vi "Test MQTT-3.1.4-2.vi"(8 "error in (no error)":errorcluster, 11 "Connection Config":refnum<class "Connection.lvclass">) -> (0 "error out":errorcluster, 3 "Connection Config dup":refnum<class "Connection.lvclass">)   [LabVIEW 2013]
uses:
  <vilib>/LabVIEW Open Source Project/MQTT Control Packets/Control Packets/CONNECT/CONNECT.lvclass
  <vilib>/LabVIEW Open Source Project/MQTT Control Packets/Control Packets/ControlPacket/ControlPacket.lvclass
  <vilib>/addons/_JKI Toolkits/Caraya/classes/Test/Test.lvclass
  <vilib>/addons/_JKI Toolkits/Caraya/classes/Assert/Assert.lvclass
  <vilib>/LabVIEW Open Source Project/MQTT Control Packets/Control Packets/DISCONNECT/DISCONNECT.lvclass
  <vilib>/LabVIEW Open Source Project/MQTT Control Packets/Control Packets/CONNACK/CONNACK.lvclass
  <vilib>/LabVIEW Open Source Project/MQTT Control Packets/Control Packets/CONNACK/Connect Return Code -- enum.ctl
  <vilib>/LabVIEW Open Source Project/Connection/Connection/Connection.lvclass
  <vilib>/LabVIEW Open Source Project/MQTT Connection/MQTT_Connection/Connection/Connection.lvclass
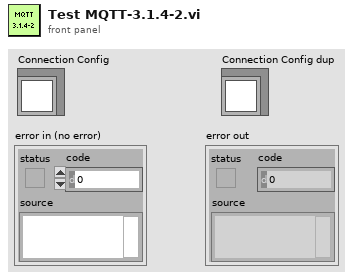
[diagram p1: front panel]
types:
  T1 = typedef "MQTT_Control_Packets.lvlib/CONNACK.lvclass/Connect Return Code -- enum.ctl" = enum16{"Connection accepted", "Unacceptable protocol version", "Identifier Rejected", "Server Unavailable", "Bad Username or Password", "Not Authorized"}
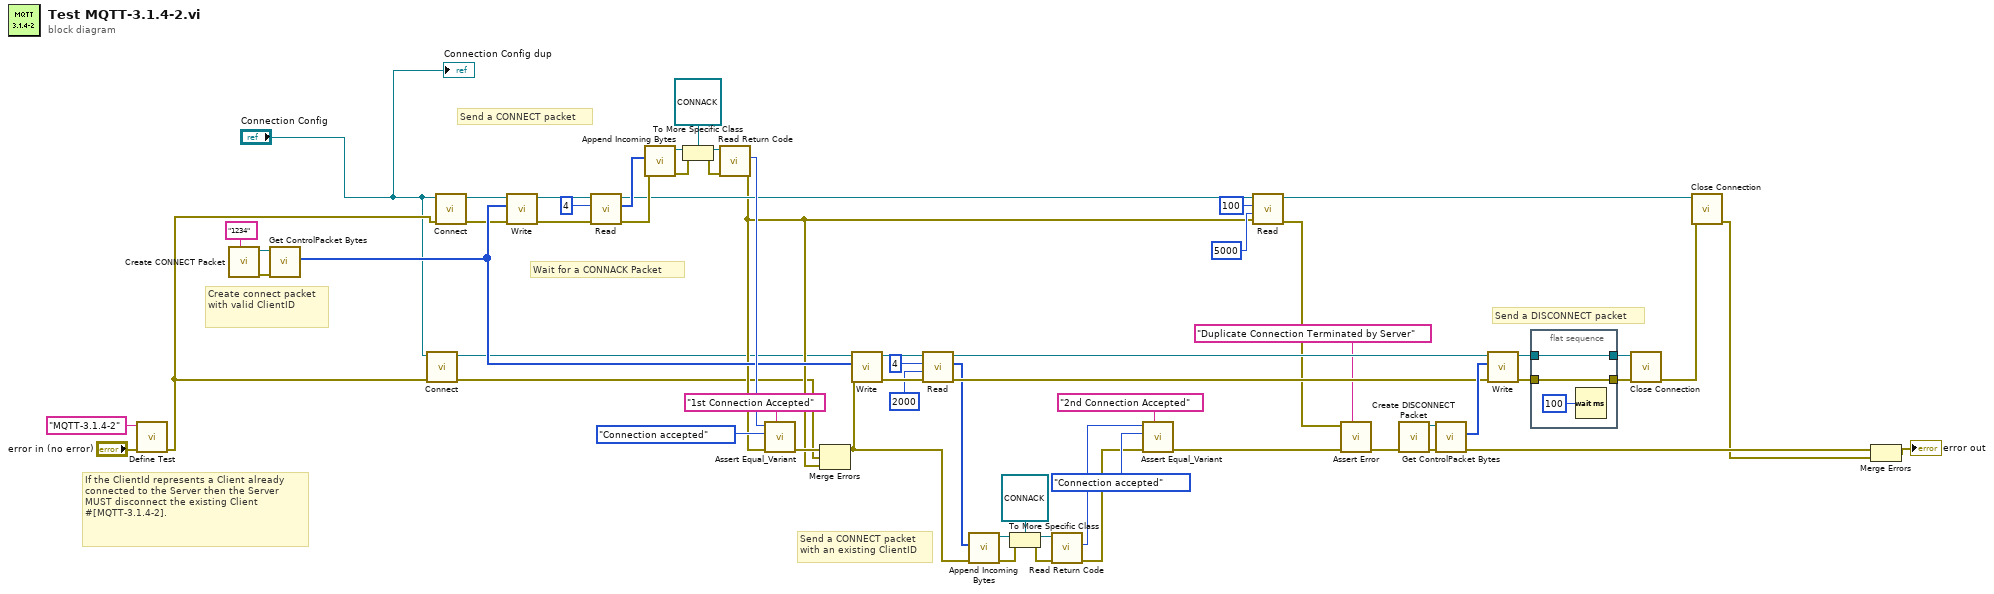
[diagram p0: block diagram]
diagram:
  # "Send a CONNECT packet\nwith an existing ClientID"
  # "If the ClientId represents a Client already connected to the Server then the Server MUST disconnect the existing Client #[MQTT-3.1.4-2]."
  # "Send a DISCONNECT packet"
  # "Wait for a CONNACK Packet"
  # "Create connect packet with valid ClientID"
  # "Send a CONNECT packet"
  n1 = call <vilib>:"Define Test.vi"("error in (no error)"="error in (no error)", "Label (VI Title)"="MQTT-3.1.4-2") -> ("error out"=w7:errorcluster)  [unwired: 9 in]
  n2 = call <vilib>:"Create CONNECT Packet.vi"("Client ID (empty: generate new)"="1234") -> ("error out"=w62:errorcluster, "CONNECT"=w63:refnum<class "CONNECT.lvclass">)  [unwired: 8 in, 1 out]
  n3 = call <vilib>:"Get ControlPacket Bytes.vi"("error in (no error)"=w62, "ControlPacket"=w63) -> ("Bytes Stream"=w38:u8[])  [unwired: 6 in, 3 out]
  n4 = call <vilib>:"Connect.vi"("error in (no error)"=w7, "Connection in"="Connection Config") -> ("error out"=w10:errorcluster, "Connection out"=w11:refnum<class "Connection.lvclass">)  [unwired: 8 in]
  n5 = call <vilib>:"Connect.vi"("error in (no error)"=w7, "Connection in"="Connection Config") -> ("error out"=w8:errorcluster, "Connection out"=w9:refnum<class "Connection.lvclass">)  [unwired: 8 in]
  n6 = call <vilib>:"Write.vi"("error in (no error)"=w8, "Bytes"=w38, "Connection in"=w9) -> ("error out"=w42:errorcluster, "Connection"=w43:refnum<class "Connection.lvclass">)  [unwired: 7 in]
  n7 = call <vilib>:"Read.vi"("error in (no error)"=w42, "bytes to read (100)"=4 ("bytes to read"), "TCPConnection in"=w43) -> ("error out"=w39:errorcluster, "Bytes"=w41:u8[], "TCPConnection out"=w28:refnum<class "Connection.lvclass">)  [unwired: 4 in, 2 out]
  n8 = call <vilib>:"Append Incoming Bytes.vi"("error in (no error)"=w39, "Incoming Packets"=w41) -> ("error out"=w45:errorcluster, "ControlPacket"=w51:refnum<class "ControlPacket.lvclass">)  [unwired: 6 in, 2 out]
  n9 = To More Specific Class(target class=refnum<class "CONNACK.lvclass"> refnum ("CONNACK"), reference=w51, error in=w45) -> (specific class reference=w50:refnum<class "CONNACK.lvclass">, error out=w46:errorcluster)
  n10 = call <vilib>:"Read Return Code.vi"("error in (no error)"=w46, "CONNACK in"=w50) -> ("error out"=w12:errorcluster, "Return Code"=w48:T1)  [unwired: 7 in, 1 out]
  n11 = call <vilib>:"Assert Equal_Variant.vi"("Label"="1st Connection Accepted", "error in (no error)"=w12, "Y"=Connect_Return_Code_--_enum."Connection accepted" ("Return Code"), "X"=w48) -> ("error out"=w27:errorcluster)  [unwired: 7 in]
  n12 = Merge Errors(w27, w10, w12) -> (w15:errorcluster)
  n13 = call <vilib>:"Write.vi"("error in (no error)"=w15, "Bytes"=w38, "Connection in"=w11) -> ("error out"=w29:errorcluster, "Connection"=w36:refnum<class "Connection.lvclass">)  [unwired: 7 in]
  n14 = call <vilib>:"Read.vi"("error in (no error)"=w29, "timeout (2000 ms)"=2000 ("timeout (1000 ms)"), "bytes to read (100)"=4 ("bytes to read"), "TCPConnection in"=w36) -> ("error out"=w30:errorcluster, "Bytes"=w24:u8[], "TCPConnection out"=w31:refnum<class "Connection.lvclass">)  [unwired: 3 in, 2 out]
  n15 = call <vilib>:"Append Incoming Bytes.vi"("error in (no error)"=w15, "Incoming Packets"=w24) -> ("error out"=w35:errorcluster, "ControlPacket"=w32:refnum<class "ControlPacket.lvclass">)  [unwired: 6 in, 2 out]
  n16 = To More Specific Class(target class=refnum<class "CONNACK.lvclass"> refnum ("CONNACK"), reference=w32, error in=w35) -> (specific class reference=w33:refnum<class "CONNACK.lvclass">, error out=w34:errorcluster)
  n17 = call <vilib>:"Read Return Code.vi"("error in (no error)"=w34, "CONNACK in"=w33) -> ("error out"=w14:errorcluster, "Return Code"=w21:T1)  [unwired: 7 in, 1 out]
  n18 = call <vilib>:"Assert Equal_Variant.vi"("Label"="2nd Connection Accepted", "error in (no error)"=w14, "Y"=Connect_Return_Code_--_enum."Connection accepted" ("Return Code"), "X"=w21) -> ("error out"=w20:errorcluster)  [unwired: 7 in]
  n19 = call <vilib>:"Read.vi"("error in (no error)"=w12, "timeout (2000 ms)"=5000 ("timeout (1000 ms)"), "bytes to read (100)"=100, "TCPConnection in"=w28) -> ("error out"=w19:errorcluster, "TCPConnection out"=w6:refnum<class "Connection.lvclass">)  [unwired: 3 in, 3 out]
  n20 = call <vilib>:"Assert Error.vi"("Label"="Duplicate Connection Terminated by Server", "error in (no error)"=w20, "Error?"=w19) -> ("error out"=w17:errorcluster)  [unwired: 8 in]
  n21 = call <vilib>:"Create DISCONNECT Packet.vi"("error in (no error)"=w17) -> ("error out"=w57:errorcluster, "DISCONNECT"=w56:refnum<class "DISCONNECT.lvclass">)  [unwired: 8 in, 1 out]
  n22 = call <vilib>:"Get ControlPacket Bytes.vi"("error in (no error)"=w57, "ControlPacket"=w56) -> ("error out"=w16:errorcluster, "Bytes Stream"=w55:u8[])  [unwired: 6 in, 2 out]
  n23 = call <vilib>:"Write.vi"("error in (no error)"=w30, "Bytes"=w55, "Connection in"=w31) -> ("error out"=w53:errorcluster, "Connection"=w54:refnum<class "Connection.lvclass">)  [unwired: 7 in]
  n24 = flat-sequence {
    tunnel: w54 -> [w66]
    tunnel: [w66] -> w52
    tunnel: [w64] -> w49
    tunnel: w53 -> [w64]
    frame #0 {
      n25 = Wait (ms)(milliseconds to wait=u32 100) -> ()  [unwired: 1 out]
    }
  }
  n26 = call <vilib>:"Close Connection.vi"("error in (no error)"=w49, "Connection in"=w52) -> ("error out"=w5:errorcluster)  [unwired: 8 in, 1 out]
  n27 = call <vilib>:"Close Connection.vi"("error in (no error)"=w5, "Connection in"=w6) -> ("error out"=w4:errorcluster)  [unwired: 8 in, 1 out]
  n28 = Merge Errors(w16, w4) -> (→"error out":errorcluster)
  "Connection Config dup" <- "Connection Config"
